vi "Get Product Name.vi"(8 "error in (no error)":errorcluster, 9 "LARGP":u32, 10 "VARIABLE":string, 11 "HANDLE":u32) -> (0 "error out":errorcluster, 2 "NOMBRE":string, 3 "SALIDA":u32)   [LabVIEW 2011, in "HID_ARZ.lvlib"]
doc: "GET_PRODUCT_NAME GetProductName;"
uses:
  HID_ARZ.lvlib
  <userlib>/HID_ARZ/mcHID.dll
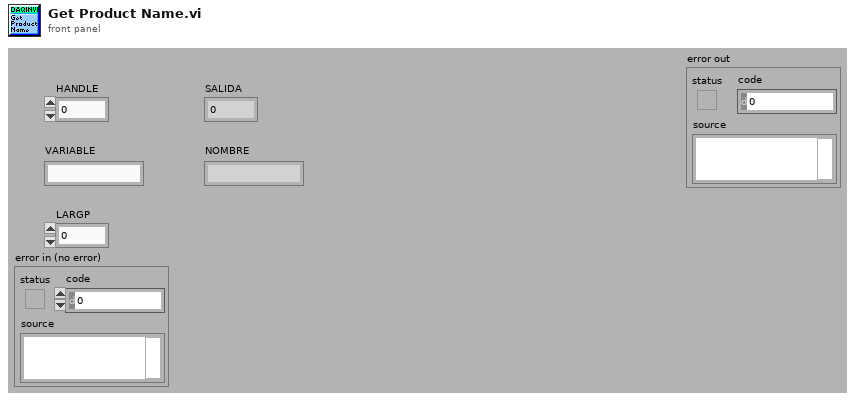
[diagram p1: front panel]
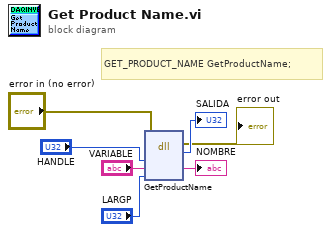
[diagram p0: block diagram]
diagram:
  # "GET_PRODUCT_NAME GetProductName;"
  n1 = dll-call lib="C:/Program Files (x86)/National Instruments/LabVIEW 2017/user.lib/HID_ARZ/mcHID.*" fn="GetProductName"(error in="error in (no error)", "para0"="HANDLE", "para1"="VARIABLE", "para2"="LARGP") -> (error out=→"error out":errorcluster, "return type"=→"SALIDA":u32, "para1"=→"NOMBRE":string)  [unwired: 4 in, 1 out]
